vi "File Path Log Action Engine.vi"(7 "Command":T1=enum."Test Procedure", 8 "error in (no error)":errorcluster, 11 "File Path In":path[](array[path])=[path "", path "", path "", path "", path ""]) -> (0 "error out":errorcluster, 3 "Read Path":path)   [LabVIEW 2021]
uses:
  Queue Test updator/Auxillary User Interface/Controls/File Path Log State Enum.ctl
  Queue Test updator/Auxillary User Interface/Controls/Path Enum Control.ctl
  <vilib>/Utility/config.llb/Write Key (Path).vi
  <vilib>/Utility/config.llb/Read Key (String).vi
  <vilib>/Utility/config.llb/Read Key (Path).vi
  <vilib>/Utility/config.llb/NI_LVConfig.lvlib
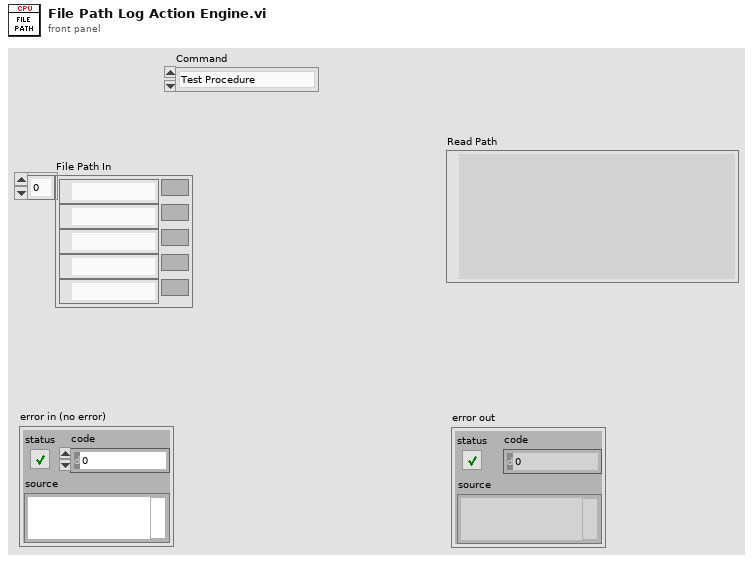
[diagram p1: front panel]
types:
  T1 = typedef "File Path Log State Enum.ctl" = enum16{"Init", "Write", "Test Procedure", "Login", "Report", "Error Log", "Action Log", "Instr. Config.", "CheckSum"}
  T2 = typedef "Path Enum Control.ctl" = enum16{"Test Procedure", "Report", "File Path", "Configuration", "Login", "Error Log", "Action Log", "Instr. Config", "Functional Command"}
  T3 = typedef "NI_LVConfig.lvlib/Config Data RefNum.ctl" = refnum<k1>
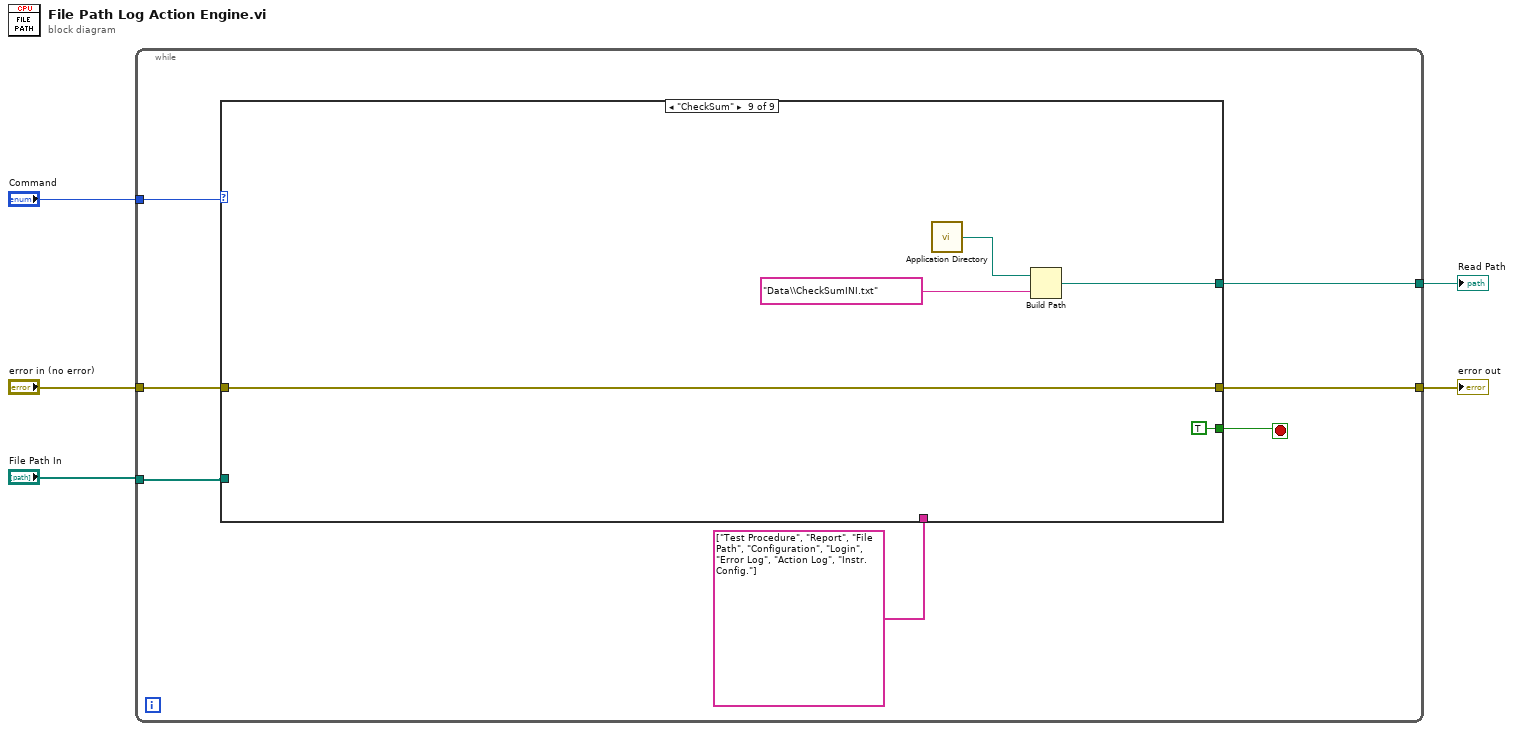
[diagram p0: block diagram]
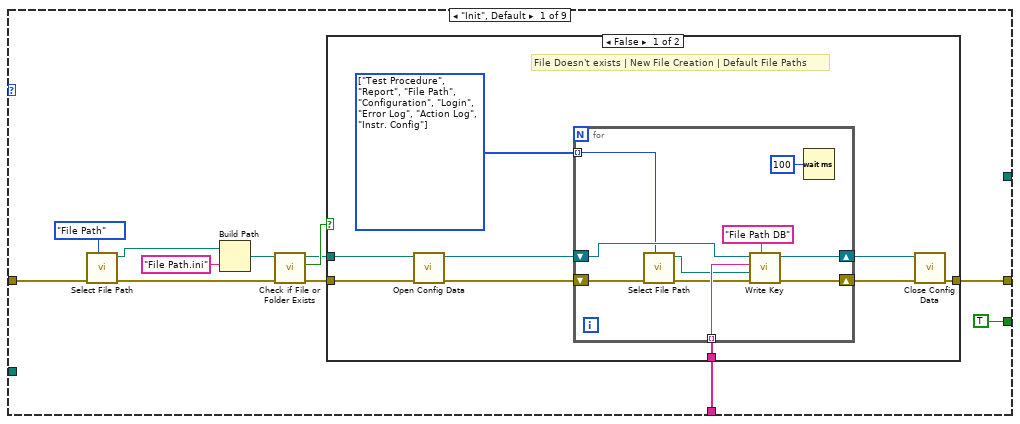
[diagram p2: hidden frame]
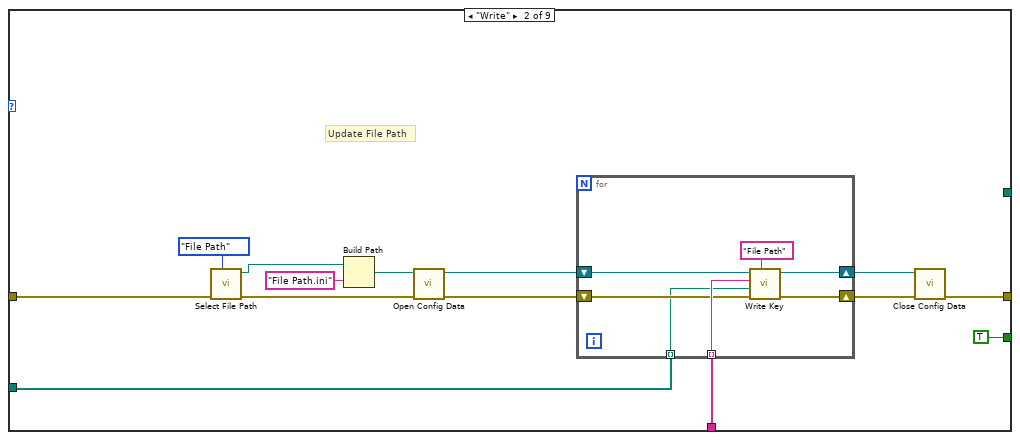
[diagram p4: hidden frame]
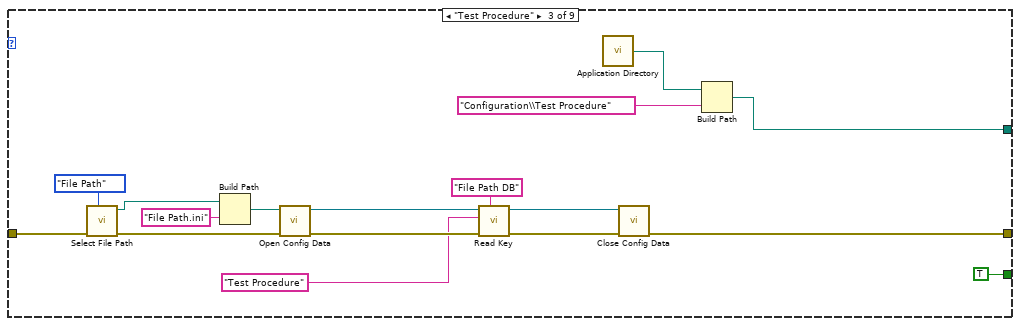
[diagram p5: hidden frame]
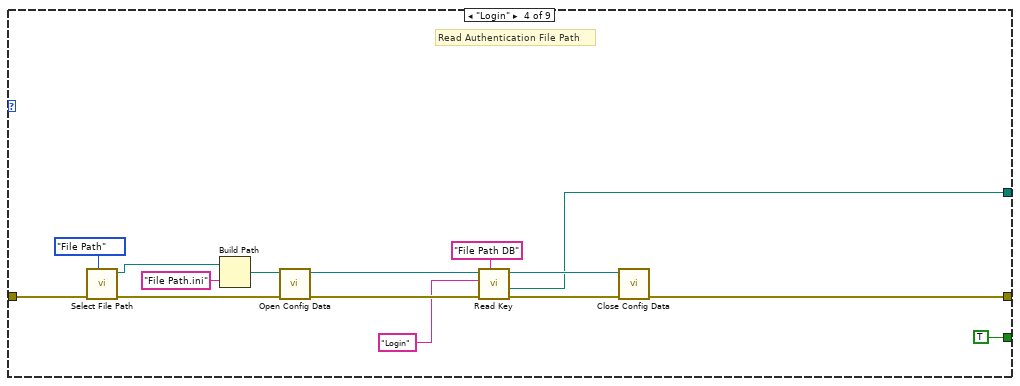
[diagram p6: hidden frame]
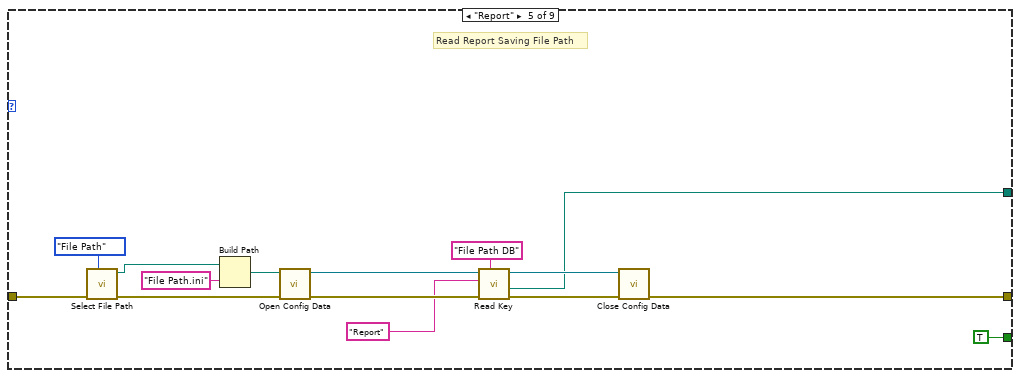
[diagram p7: hidden frame]
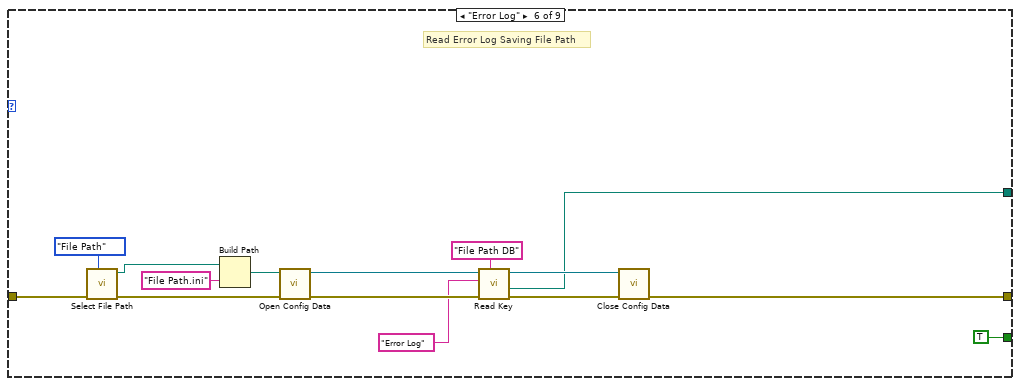
[diagram p8: hidden frame]
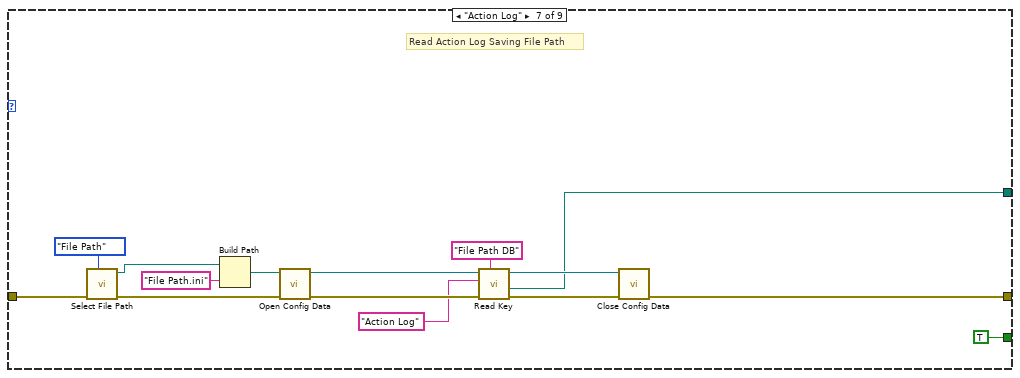
[diagram p9: hidden frame]
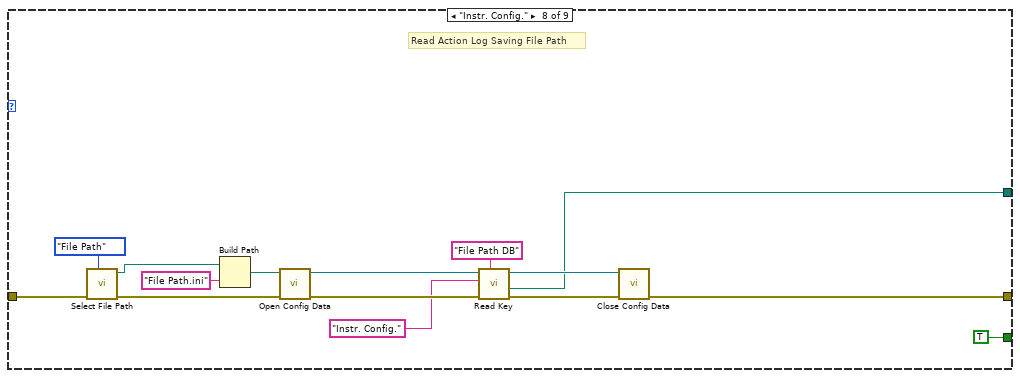
[diagram p10: hidden frame]
diagram:
  n1 = while {
    tunnel: "Command" -> [w12]
    tunnel: "error in (no error)" -> [w11]
    tunnel: [w10] -> w3
    tunnel: [w7] -> w2
    tunnel: "File Path In" -> [w6]
    stop <- w8 stop-if-true
    n2 = case shown="\"CheckSum\"" w12 {
      tunnel: w11 -> [w23 w46 w81 w96 w111 w126 w141 w156 w162]
      tunnel: [w21 w58 w79 w94 w109 w124 w139 w154 w162] -> w10
      tunnel: string[] ["Test Procedure", "Report", "File Path", "Configuration", "Login", "Error Log", "Action Log", "Instr. Config."] ("name or relative path") -> [w14 w57 _ _ _ _ _ _ _]
      tunnel: [TRUE TRUE TRUE TRUE TRUE TRUE TRUE TRUE TRUE] -> w8
      tunnel: [_ _ w67 w83 w98 w113 w128 w143 w158] -> w7
      tunnel: w6 -> [_ w51 _ _ _ _ _ _ _]
      frame "Init", Default {
        n3 = call "Select File Path.vi"("Command"=Path_Enum_Control."File Path", "error in (no error)"=w23) -> ("error out"=w22:errorcluster, "Path Out"=w20:path)  [unwired: 8 in]
        n4 = Build Path(base path=w20, name or relative path="File Path.ini") -> (appended path=w17:path)
        n5 = call <vilib>:"Check if File or Folder Exists.vi"("error in (no error)"=w22, "path"=w17) -> ("error out"=w18:errorcluster, "file or folder exists?"=w16:bool, "dup path"=w15:path)  [unwired: 7 in]
        n6 = case shown="False" w16 {
          tunnel: [w27 w44] -> w21
          tunnel: w18 -> [w32 w44]
          tunnel: w15 -> [w31 _]
          tunnel: w14 -> [w29 _]
          frame False {
            w25 = T2[] [enum."Test Procedure", enum."Report", enum."File Path", enum."Configuration", enum."Login", enum."Error Log", enum."Action Log", enum."Instr. Config"] items=["Test Procedure", "Report", "File Path", "Configuration", "Login", "Error Log", "Action Log", "Instr. Config", "Functional Command"] ("Array")
            # "File Doesn't exists | New File Creation | Default File Paths"
            n7 = call <vilib>:"Open Config Data.vi"("error in (no error)"=w32, "configuration file path"=w31) -> ("error out"=w33:errorcluster, "refnum"=w30:T3)  [unwired: 7 in, 1 out]
            n8 = for {
              shift-right: [w36] -> w26
              shift-left: w33 -> [w43]
              tunnel: w29 -> [w40] mode=indexing
              shift-right: [w37] -> w28
              shift-left: w30 -> [w42]
              tunnel: w25 -> [w34] mode=indexing
              n9 = call "Select File Path.vi"("Command"=w34, "error in (no error)"=w43) -> ("error out"=w39:errorcluster, "Path Out"=w38:path)  [unwired: 8 in]
              n10 = call-poly <vilib>:"Write Key.vi"("section"="File Path DB" ("name or relative path"), "error in (no error)"=w39, "value"=w38, "key"=w40, "refnum"=w42) -> ("error out"=w36:errorcluster, "refnum out"=w37:T3)  [unwired: 4 in, 1 out]
              n11 = Wait (ms)(milliseconds to wait=u32 100) -> ()  [unwired: 1 out]
            }
            n12 = call <vilib>:"Close Config Data.vi"("error in (no error)"=w26, "refnum"=w28) -> ("error out"=w27:errorcluster)  [unwired: 8 in, 1 out]
          }
          frame True {
            # "File Already Exists"
          }
        }
      }
      frame "Write" {
        # "Update File Path"
        n13 = call "Select File Path.vi"("Command"=Path_Enum_Control."File Path", "error in (no error)"=w46) -> ("error out"=w45:errorcluster, "Path Out"=w49:path)  [unwired: 8 in]
        n14 = Build Path(base path=w49, name or relative path="File Path.ini") -> (appended path=w47:path)
        n15 = call <vilib>:"Open Config Data.vi"("error in (no error)"=w45, "configuration file path"=w47) -> ("error out"=w55:errorcluster, "refnum"=w54:T3)  [unwired: 7 in, 1 out]
        n16 = for {
          shift-right: [w61] -> w52
          shift-left: w55 -> [w60]
          tunnel: w57 -> [w63] mode=indexing
          shift-right: [w62] -> w53
          shift-left: w54 -> [w65]
          tunnel: w51 -> [w59] mode=indexing
          n17 = call-poly <vilib>:"Write Key.vi"("section"="File Path" ("name or relative path"), "error in (no error)"=w60, "value"=w59, "key"=w63, "refnum"=w65) -> ("error out"=w61:errorcluster, "refnum out"=w62:T3)  [unwired: 4 in, 1 out]
        }
        n18 = call <vilib>:"Close Config Data.vi"("error in (no error)"=w52, "refnum"=w53) -> ("error out"=w58:errorcluster)  [unwired: 8 in, 1 out]
      }
      frame "Test Procedure" {
        n19 = call "Select File Path.vi"("Command"=Path_Enum_Control."File Path", "error in (no error)"=w81) -> ("error out"=w80:errorcluster, "Path Out"=w78:path)  [unwired: 8 in]
        n20 = Build Path(base path=w78, name or relative path="File Path.ini") -> (appended path=w76:path)
        n21 = call <vilib>:"Open Config Data.vi"("error in (no error)"=w80, "configuration file path"=w76) -> ("error out"=w74:errorcluster, "refnum"=w73:T3)  [unwired: 7 in, 1 out]
        n22 = call-poly <vilib>:"Read Key.vi"("section"="File Path DB" ("name or relative path"), "error in (no error)"=w74, "key"="Test Procedure" ("name or relative path"), "refnum"=w73) -> ("error out"=w71:errorcluster, "refnum out"=w72:T3)  [unwired: 4 in, 2 out]
        n23 = call <vilib>:"Application Directory.vi"() -> ("Application Directory"=w68:path)
        n24 = call <vilib>:"Close Config Data.vi"("error in (no error)"=w71, "refnum"=w72) -> ("error out"=w79:errorcluster)  [unwired: 8 in, 1 out]
        n25 = Build Path(base path=w68, name or relative path="Configuration\\Test Procedure") -> (appended path=w67:path)
      }
      frame "Login" {
        # "Read Authentication File Path"
        n26 = call "Select File Path.vi"("Command"=Path_Enum_Control."File Path", "error in (no error)"=w96) -> ("error out"=w95:errorcluster, "Path Out"=w93:path)  [unwired: 8 in]
        n27 = Build Path(base path=w93, name or relative path="File Path.ini") -> (appended path=w91:path)
        n28 = call <vilib>:"Open Config Data.vi"("error in (no error)"=w95, "configuration file path"=w91) -> ("error out"=w89:errorcluster, "refnum"=w88:T3)  [unwired: 7 in, 1 out]
        n29 = call-poly <vilib>:"Read Key.vi"("section"="File Path DB" ("name or relative path"), "error in (no error)"=w89, "key"="Login" ("name or relative path"), "refnum"=w88) -> ("error out"=w86:errorcluster, "value"=w83:path, "refnum out"=w87:T3)  [unwired: 4 in, 1 out]
        n30 = call <vilib>:"Close Config Data.vi"("error in (no error)"=w86, "refnum"=w87) -> ("error out"=w94:errorcluster)  [unwired: 8 in, 1 out]
      }
      frame "Report" {
        # "Read Report Saving File Path"
        n31 = call "Select File Path.vi"("Command"=Path_Enum_Control."File Path", "error in (no error)"=w111) -> ("error out"=w110:errorcluster, "Path Out"=w108:path)  [unwired: 8 in]
        n32 = Build Path(base path=w108, name or relative path="File Path.ini") -> (appended path=w106:path)
        n33 = call <vilib>:"Open Config Data.vi"("error in (no error)"=w110, "configuration file path"=w106) -> ("error out"=w104:errorcluster, "refnum"=w103:T3)  [unwired: 7 in, 1 out]
        n34 = call-poly <vilib>:"Read Key.vi"("section"="File Path DB" ("name or relative path"), "error in (no error)"=w104, "key"="Report" ("name or relative path"), "refnum"=w103) -> ("error out"=w101:errorcluster, "value"=w98:path, "refnum out"=w102:T3)  [unwired: 4 in, 1 out]
        n35 = call <vilib>:"Close Config Data.vi"("error in (no error)"=w101, "refnum"=w102) -> ("error out"=w109:errorcluster)  [unwired: 8 in, 1 out]
      }
      frame "Error Log" {
        # "Read Error Log Saving File Path"
        n36 = call "Select File Path.vi"("Command"=Path_Enum_Control."File Path", "error in (no error)"=w126) -> ("error out"=w125:errorcluster, "Path Out"=w123:path)  [unwired: 8 in]
        n37 = Build Path(base path=w123, name or relative path="File Path.ini") -> (appended path=w121:path)
        n38 = call <vilib>:"Open Config Data.vi"("error in (no error)"=w125, "configuration file path"=w121) -> ("error out"=w119:errorcluster, "refnum"=w118:T3)  [unwired: 7 in, 1 out]
        n39 = call-poly <vilib>:"Read Key.vi"("section"="File Path DB" ("name or relative path"), "error in (no error)"=w119, "key"="Error Log" ("name or relative path"), "refnum"=w118) -> ("error out"=w116:errorcluster, "value"=w113:path, "refnum out"=w117:T3)  [unwired: 4 in, 1 out]
        n40 = call <vilib>:"Close Config Data.vi"("error in (no error)"=w116, "refnum"=w117) -> ("error out"=w124:errorcluster)  [unwired: 8 in, 1 out]
      }
      frame "Action Log" {
        # "Read Action Log Saving File Path"
        n41 = call "Select File Path.vi"("Command"=Path_Enum_Control."File Path", "error in (no error)"=w141) -> ("error out"=w140:errorcluster, "Path Out"=w138:path)  [unwired: 8 in]
        n42 = Build Path(base path=w138, name or relative path="File Path.ini") -> (appended path=w136:path)
        n43 = call <vilib>:"Open Config Data.vi"("error in (no error)"=w140, "configuration file path"=w136) -> ("error out"=w134:errorcluster, "refnum"=w133:T3)  [unwired: 7 in, 1 out]
        n44 = call-poly <vilib>:"Read Key.vi"("section"="File Path DB" ("name or relative path"), "error in (no error)"=w134, "key"="Action Log" ("name or relative path"), "refnum"=w133) -> ("error out"=w131:errorcluster, "value"=w128:path, "refnum out"=w132:T3)  [unwired: 4 in, 1 out]
        n45 = call <vilib>:"Close Config Data.vi"("error in (no error)"=w131, "refnum"=w132) -> ("error out"=w139:errorcluster)  [unwired: 8 in, 1 out]
      }
      frame "Instr. Config." {
        # "Read Action Log Saving File Path"
        n46 = call "Select File Path.vi"("Command"=Path_Enum_Control."File Path", "error in (no error)"=w156) -> ("error out"=w155:errorcluster, "Path Out"=w153:path)  [unwired: 8 in]
        n47 = Build Path(base path=w153, name or relative path="File Path.ini") -> (appended path=w151:path)
        n48 = call <vilib>:"Open Config Data.vi"("error in (no error)"=w155, "configuration file path"=w151) -> ("error out"=w149:errorcluster, "refnum"=w148:T3)  [unwired: 7 in, 1 out]
        n49 = call-poly <vilib>:"Read Key.vi"("section"="File Path DB" ("name or relative path"), "error in (no error)"=w149, "key"="Instr. Config." ("name or relative path"), "refnum"=w148) -> ("error out"=w146:errorcluster, "value"=w143:path, "refnum out"=w147:T3)  [unwired: 4 in, 1 out]
        n50 = call <vilib>:"Close Config Data.vi"("error in (no error)"=w146, "refnum"=w147) -> ("error out"=w154:errorcluster)  [unwired: 8 in, 1 out]
      }
      frame "CheckSum" {
        n51 = call <vilib>:"Application Directory.vi"() -> ("Application Directory"=w160:path)
        n52 = Build Path(base path=w160, name or relative path="Data\\CheckSumINI.txt") -> (appended path=w158:path)
      }
    }
  }
  "error out" <- w3
  "Read Path" <- w2
